vi "FiniteAdd.vi"() -> ()   [LabVIEW 2024]
panel:
  out "Sum":dbl
  in  "B":dbl=3.0
  in  "A":dbl=2.0
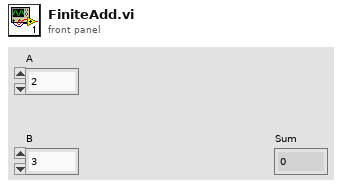
[diagram p1: front panel]
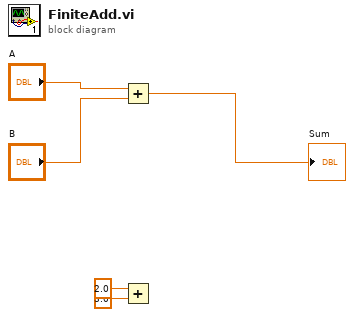
[diagram p0: block diagram]
diagram:
  n1 = Add(x="A", y="B") -> (x+y=→"Sum":dbl)
  n2 = Add(x=2.0, y=3.0) -> ()  [unwired: 1 out]
